vi "RemoteVI Test Hex To Bytes.vi"(0 "hex":string) -> (4 "bytes":string)   [LabVIEW 2020]
doc: "Test support: decodes a lowercase hex string (as written in tests/vectors) into the bytes it stands for. Two hex digits per byte; digits 0-9 and a-f. Pure."
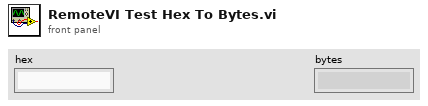
[diagram p1: front panel]
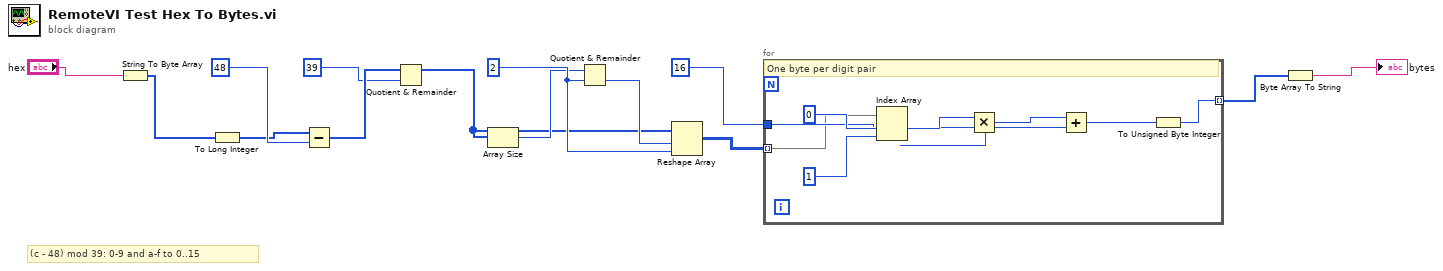
[diagram p0: block diagram]
diagram:
  w10 = 2
  # "(c - 48) mod 39: 0-9 and a-f to 0..15"
  n1 = String To Byte Array(string="hex") -> (unsigned byte array=w2:u8[])
  n2 = To Long Integer(number=w2) -> (32bit integer=w3:i32[])
  n3 = Subtract(x=w3, y=48) -> (x-y=w7:i32[])
  n4 = Quotient & Remainder(x=w7, y=39) -> (x-y*floor(x/y)=w8:i32[])  [unwired: 1 out]
  n5 = Array Size(array=w8) -> (size(s)=w9:i32)
  n6 = Quotient & Remainder(x=w9, y=w10) -> (floor(x/y)=w11:i32)  [unwired: 1 out]
  n7 = Reshape Array(w8, w11, w10) -> (w12:i32[][])
  n8 = for {
    tunnel: 16 -> [w16]
    tunnel: w12 -> [w15] mode=indexing
    tunnel: [w23] -> w13 mode=indexing
    # "One byte per digit pair"
    n9 = Index Array(array=w15, index #1=0, index #2=1) -> (element #1=w19:i32, element #2=w20:i32)
    n10 = Multiply(x=w19, y=w16) -> (x*y=w21:i32)
    n11 = Add(x=w21, y=w20) -> (x+y=w22:i32)
    n12 = To Unsigned Byte Integer(number=w22) -> (unsigned 8bit integer=w23:u8)
  }
  n13 = Byte Array To String(unsigned byte array=w13) -> (string=→"bytes":string)
